vi "VirtualATE.vi"() -> ()   [LabVIEW 2026]
uses:
  <vilib>/NI/Modbus Library/API/Modbus API.lvclass/Modbus API.ctl
  <vilib>/NI/Modbus Library/Transmission Data Unit/Transmission Data Unit.lvclass/Transmission Data Unit.ctl
  <vilib>/NI/Modbus Library/Transmission Data Unit/Write Unit ID.vi
  <vilib>/NI/Modbus Library/API/Read Transmission Data Unit.vi
  <vilib>/NI/Modbus Library/API/Write Transmission Data Unit.vi
  <vilib>/NI/Modbus Library/API/Master/Modbus Master.lvclass
  <vilib>/NI/Modbus Library/API/Wrapper/Create TCP Master.vi
  <vilib>/NI/Modbus Library/API/Wrapper/API Main.lvlib
panel:
  in  "ATE 읽기 정지":bool
  out "ALARM_CODE":u16
  out "SEQ_STATE":u16
  out "TEEST_RESULT_LATCH":u16
  out "ATE_DONE":u16
  out "ATE_RESPONSE_ID":u16
  out "ATE_RESULT":u16
  out "ATE_REQUEST_ID":u16
  out "ATE_REQUEST":u16
  out "마지막 Modbus 읽기 정상":bool
  out "수신 레지스터":u16[](array[numeric])
  out "error out":errorcluster
  in  "Unit ID":u8
  in  "Port":u16
  in  "Server IP":string
  # "0 ATE_LINK_TEST\n1 ATE_REQUEST\n2 ATE_REQUEST_ID\n3 ATE_RESULT\n4 ATE_RESPONSE_ID\n5 ATE_DONE\n6 TEST_RESULT_LATCH\n7 SEQ_STATE\n8 ALARM_CODE"
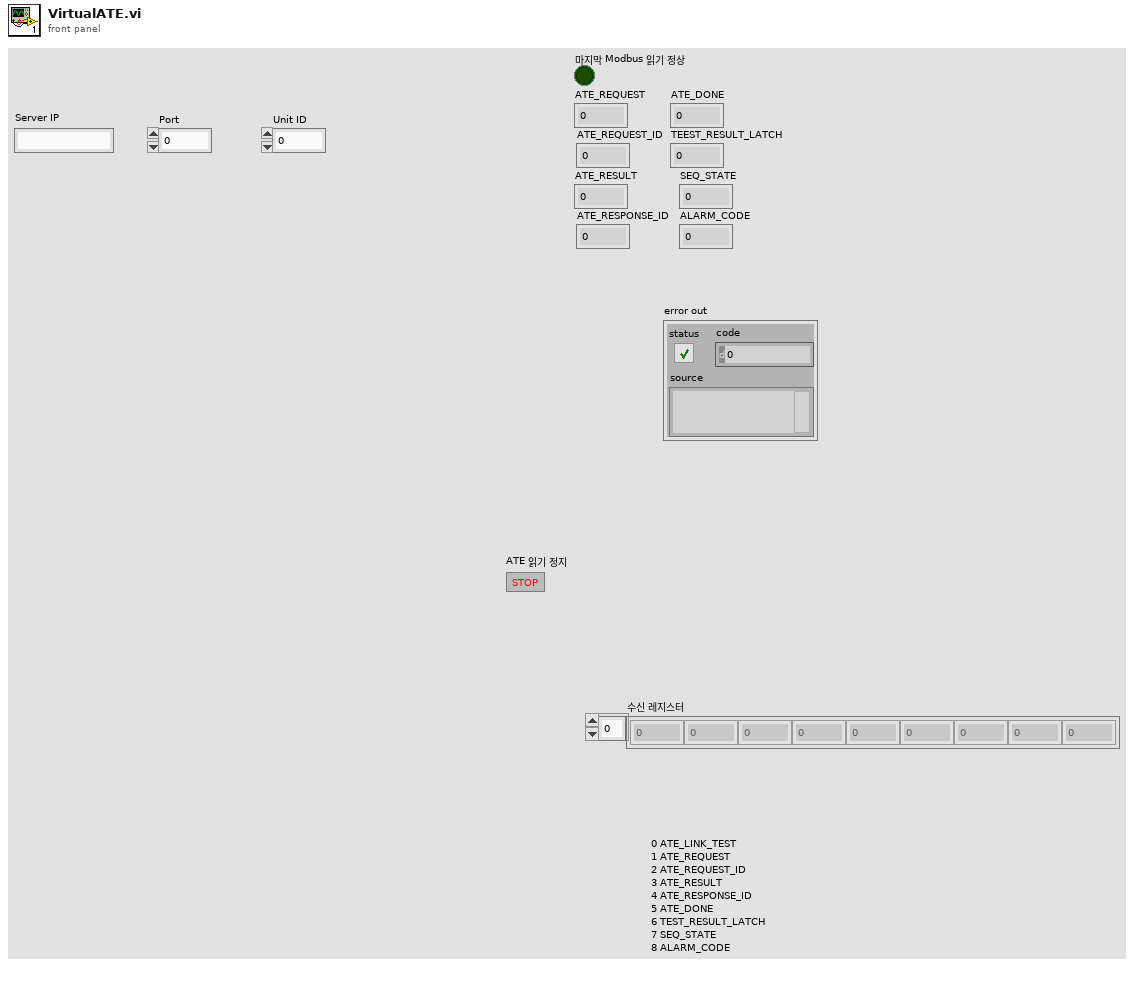
[diagram p1: front panel]
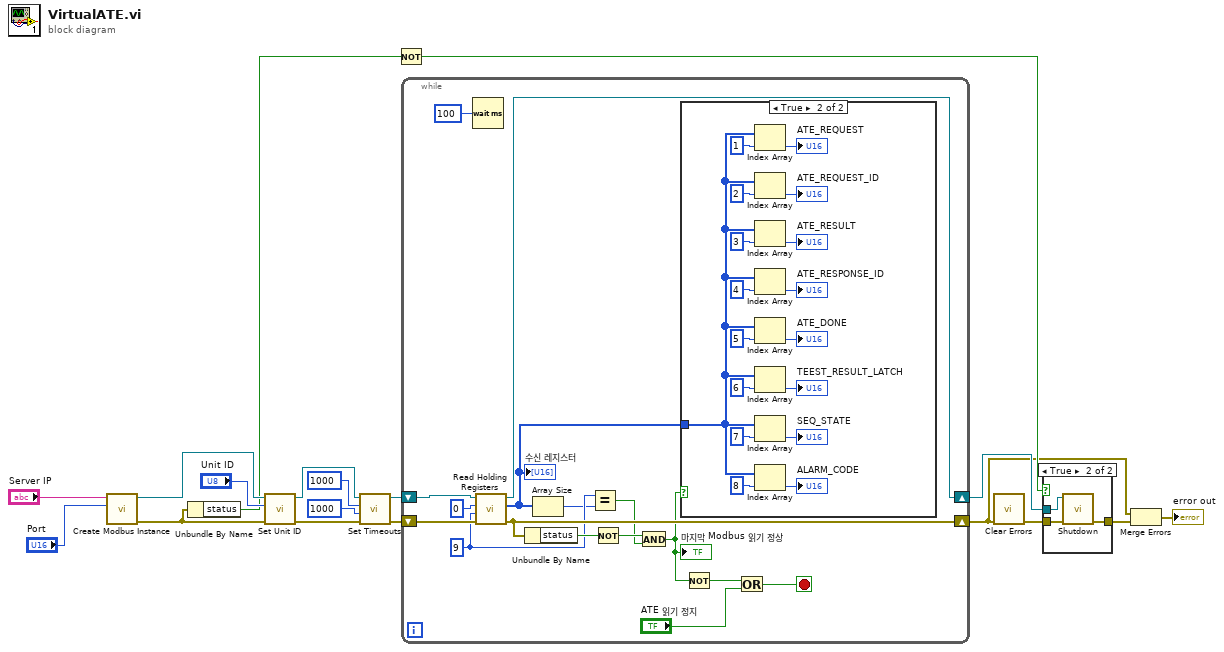
[diagram p0: block diagram]
diagram:
  n1 = call-poly <vilib>:"Create Modbus Instance.vi"("port (502)"="Port", "address"="Server IP") -> ("error out"=w8:errorcluster, "TCP master instance"=w13:refnum<class "Modbus Master.lvclass">)  [unwired: 8 in]
  n2 = Unbundle By Name(w8) -> ("status"=w7:bool)
  n3 = call <vilib>:"Set Unit ID.vi"("error in"=w8, "unit ID"="Unit ID", "Modbus master in"=w13) -> ("error out"=w11:errorcluster, "Modbus master out"=w12:refnum<class "Modbus Master.lvclass">)  [unwired: 7 in]
  n4 = call <vilib>:"Set Timeouts.vi"("error in"=w11, "write operation timeout"=1000, "read operation timeout"=1000, "Modbus master in"=w12) -> ("error out"=w9:errorcluster, "Modbus master out"=w10:refnum<class "Modbus Master.lvclass">)  [unwired: 6 in]
  n5 = Not(x=w7) -> (.not. x?=w6:bool)
  n6 = while {
    shift-right: [w29] -> w2
    shift-left: w9 -> [w30]
    shift-right: [w31] -> w5
    shift-left: w10 -> [w32]
    stop <- w19 stop-if-true
    w27 = u16 9 ("number of inputs")
    n7 = Wait (ms)(milliseconds to wait=u32 100) -> ()  [unwired: 1 out]
    n8 = call-dynamic "Read Holding Registers.vi"("error in"=w30, "number of inputs"=w27, "starting address"=u16 0, "Modbus master in"=w32) -> ("error out"=w29:errorcluster, "register values"=w23:u16[], "Modbus master out"=w31:refnum<class "Modbus Master.lvclass">)  [unwired: 5 in]
    "수신 레지스터" <- w23
    n9 = Unbundle By Name(w29) -> ("status"=w28:bool)
    n10 = Array Size(array=w23) -> (size(s)=w26:i32)
    n11 = Equal?(x=w27, y=w26) -> (x = y?=w24:bool)
    n12 = Not(x=w28) -> (.not. x?=w25:bool)
    n13 = And(x=w25, y=w24) -> (x .and. y?=w22:bool)
    "마지막 Modbus 읽기 정상" <- w22
    n14 = case shown="True" w22 {
      tunnel: w23 -> [_ w49]
      frame False {
      }
      frame True {
        n15 = Index Array(array=w49, index=1) -> (element=→"ATE_REQUEST":u16)
        n16 = Index Array(array=w49, index=2) -> (element=→"ATE_REQUEST_ID":u16)
        n17 = Index Array(array=w49, index=3) -> (element=→"ATE_RESULT":u16)
        n18 = Index Array(array=w49, index=4) -> (element=→"ATE_RESPONSE_ID":u16)
        n19 = Index Array(array=w49, index=5) -> (element=→"ATE_DONE":u16)
        n20 = Index Array(array=w49, index=6) -> (element=→"TEEST_RESULT_LATCH":u16)
        n21 = Index Array(array=w49, index=7) -> (element=→"SEQ_STATE":u16)
        n22 = Index Array(array=w49, index=8) -> (element=→"ALARM_CODE":u16)
      }
    }
    n23 = Not(x=w22) -> (.not. x?=w21:bool)
    n24 = Or(x=w21, y="ATE 읽기 정지") -> (x .or. y?=w19:bool)
  }
  n25 = call <vilib>:"Clear Errors.vi"("error in (no error)"=w2) -> ("error out"=w1:errorcluster)  [unwired: 5 in, 1 out]
  n26 = case shown="True" w6 {
    tunnel: w5 -> [_ w55]
    tunnel: [w52 w54] -> w4
    tunnel: w1 -> [w52 w53]
    frame False {
    }
    frame True {
      n27 = call-dynamic "Shutdown.vi"("error in"=w53, "Modbus master in"=w55) -> ("error out"=w54:errorcluster)  [unwired: 9 in]
    }
  }
  n28 = Merge Errors(w2, w4) -> (→"error out":errorcluster)
